vi "Scheduler_Advance.vi"(8 "error in (no error)":errorcluster={"status"=FALSE, "code"=0, "source"="\"\""}, 10 "execution graph":string, 11 "Step completion event":string) -> (0 "error out":errorcluster={"status"=FALSE, "code"=0, "source"="\"\""}, 2 "status ok":bool, 3 "New ready nodes/group status":string)   [LabVIEW 2026]
doc: "INTENT: Update graph execution and results. LOGIC: Commit action terminal status, update dependency counters, queue next actions or cycle boundary."
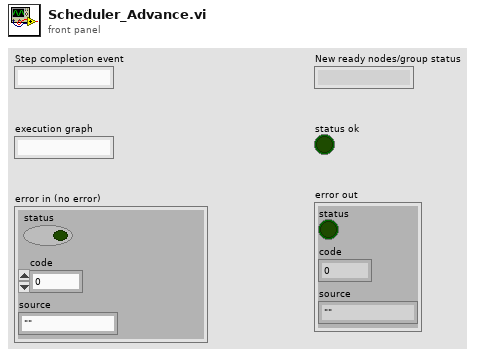
[diagram p1: front panel]
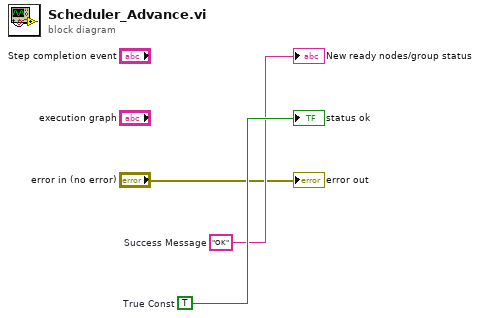
[diagram p0: block diagram]
diagram:
  w3 = TRUE  # True Const
  w2 = "OK"  # Success Message
  "New ready nodes/group status" <- w2
  "status ok" <- w3
  "error out" <- "error in (no error)"
